vi "[ce] Partial Derivatives of f(x1,x2).vi"(5 "derivative":u16(ring) items=["first variable", "second variable"], 6 "parameters":cluster{"name":string, "value":dbl}[](array[cluster]) {"value" format="%.2f"}, 7 "# points":u32=25, 8 "error in":errorcluster, 9 "formula info":T1={"formula"="", "variable 1"="x1", "variable 2"="x2"}, 10 "End":cluster{"x1":dbl, "x2":dbl}={"x1"=1.0, "x2"=1.0} {"x2" format="%.2f"; "x1" format="%.2f"}, 11 "Start":cluster{"x1":dbl, "x2":dbl} {"x2" format="%.2f"; "x1" format="%.2f"}) -> (0 "error out":errorcluster, 1 "Partial derivative of f(x1,x2)":dbl[][](array[numeric]) format="%.2f", 2 "X2  Values":dbl[](array[numeric]) format="%.2f", 3 "X1 Values":dbl[](array[numeric]) format="%.2f", 4 "ticks":u32)   [LabVIEW 2021]
doc: "Calculates a 2D array of the partial derivatives of a function of two independent variables.\nThe VI allows specifying additional parameters and evaluating them in formula.\n\n::: CalcExpress Toolkit :::\nCopyright (c) 2000-2026 Konstantin Shifershteyn. All rights reserved."
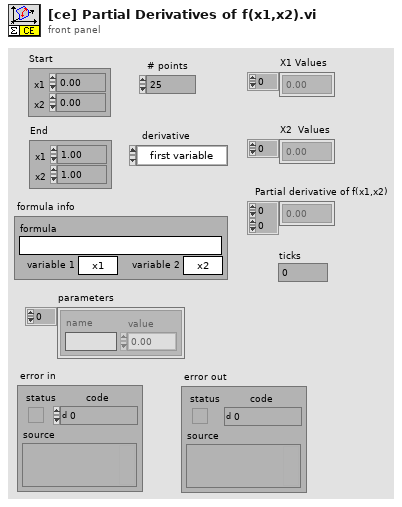
[diagram p1: front panel]
types:
  T1 = cluster{"formula":string, "variable 1":string, "variable 2":string}
  T2 = enum16{"create", "destroy", "set value", "get value"}
  T3 = typedef "VarMan Variable Context Handle.ctl" = i32
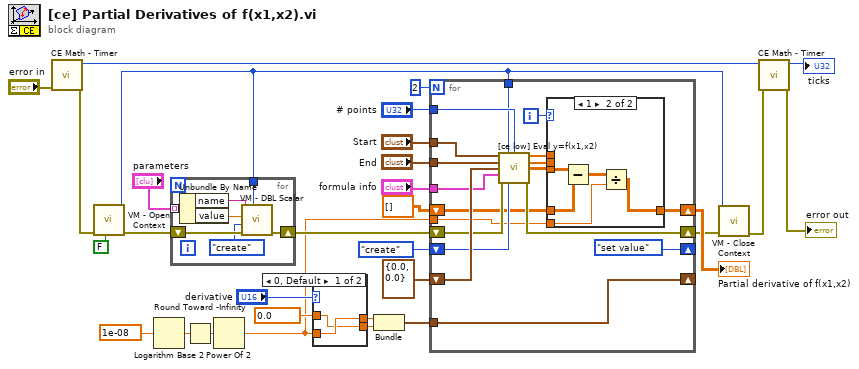
[diagram p0: block diagram]
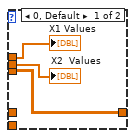
[diagram p2: hidden frame]
diagram:
  n1 = call "CE Math - Timer.vi"("error in (no error)"="error in") -> ("error out"=w30:errorcluster, "ticks out"=w28:u32)  [unwired: 7 in]
  n2 = call "VM - Open Context.vi"("close loose contexts (F)"=FALSE ("close loose contexts (T)"), "error in"=w30) -> ("error out"=w24:errorcluster, "VC Handle out"=w7:T3)  [unwired: 7 in, 1 out]
  n3 = Logarithm Base 2(1:1e-08 ("h")) -> (0:w5:dbl)
  n4 = for {
    shift-right: [w34] -> w9
    shift-left: w24 -> [w35]
    tunnel: "parameters" -> [w32] mode=indexing
    tunnel: w7 -> [w31]
    n5 = Unbundle By Name(w32) -> ("name"=w36:string, "value"=w37:dbl)
    n6 = call "VM - DBL Scalar.vi"("VC Handle"=w31, "error in"=w35, "cmd"=T2."create", "value in"=w37, "name_spec"=w36) -> ("error out"=w34:errorcluster)  [unwired: 1 in, 5 out]
  }
  n7 = Round Toward -Infinity(1:w5) -> (0:w4:dbl)
  n8 = Power Of 2(x=w4) -> (2^x=w2:dbl)
  n9 = case shown="0, Default" "derivative" {
    tunnel: 0.0 ("h") -> [w38 w41]
    tunnel: [w39 w41] -> w21
    tunnel: w2 -> [w39 w40]
    tunnel: [w38 w40] -> w20
    frame 0, Default {
    }
    frame 1 {
    }
  }
  n10 = Bundle("h"=w21, "h"=w20) -> (w18:cluster{"h":dbl, "h":dbl})  [unwired: 1 in]
  n11 = for {
    N: 2 -> [_]
    shift-right: [w56] -> w10
    shift-left: w9 -> [w57]
    shift-right: [T2."set value" ("vm cmd")] -> _
    shift-left: T2."create" ("vm cmd") -> [w55]
    shift-right: [w58] -> _
    shift-left: cluster{"h":dbl, "h":dbl} {"h"=0.0, "h"=0.0} -> [w59]
    tunnel: w18 -> [w58]
    tunnel: "formula info" -> [w53]
    tunnel: "End" -> [w52]
    tunnel: "Start" -> [w51]
    shift-right: [w49] -> w14
    shift-left: dbl[][] [] ("Y Values") -> [w46]
    tunnel: w2 -> [w45]
    tunnel: "# points" -> [w44]
    tunnel: w7 -> [w43]
    i -> [w50]
    n12 = call "[ce low] Eval y=f(x1,x2).vi"("Start"=w51, "VC Handle"=w43, "number of points"=w44, "End"=w52, "offset"=w59, "formula info"=w53, "error in"=w57, "vm cmd"=w55) -> ("X1 Values"=w48:dbl[], "X2  Values"=w47:dbl[], "Y Values"=w42:dbl[][], "error out"=w56:errorcluster)  [unwired: 4 in]
    n13 = case shown="1" w50 {
      tunnel: [w62 w64] -> w49
      tunnel: w42 -> [w62 w66]
      tunnel: w48 -> [w61 _]
      tunnel: w47 -> [w60 _]
      tunnel: w46 -> [_ w65]
      tunnel: w45 -> [_ w63]
      frame 0, Default {
        "X1 Values" <- w61
        "X2  Values" <- w60
      }
      frame 1 {
        n14 = Subtract(x=w66, y=w65) -> (x-y=w67:dbl[][])
        n15 = Divide(x=w67, y=w63) -> (x/y=w64:dbl[][])
      }
    }
  }
  "Partial derivative of f(x1,x2)" <- w14
  n16 = call "VM - Close Context.vi"("error in"=w10, "VC Handle"=w7) -> ("error out"=w29:errorcluster)  [unwired: 8 in, 1 out]
  n17 = call "CE Math - Timer.vi"("error in (no error)"=w29, "ticks in"=w28) -> ("error out"=→"error out":errorcluster, "ticks out"=→"ticks":u32)  [unwired: 6 in]
